vi "W07_Count.vi"() -> ()   [LabVIEW 2018]
doc: "Use this template to build a VI to use as a subVI."
panel:
  in  "stop":bool
  in  "sim read fails":bool
  in  "sim rate per s":u16
  in  "sim start":u16
  out "total this shift":u32
  out "this second":u16
  out "D202":u16
  in  "VISA resource (PLC)":refnum<visa-resource-name>
  # "FX_ReadD.vi here is a fake (W07_sub). Set sim start 65530 and sim rate 3 to see the U16 wrap."
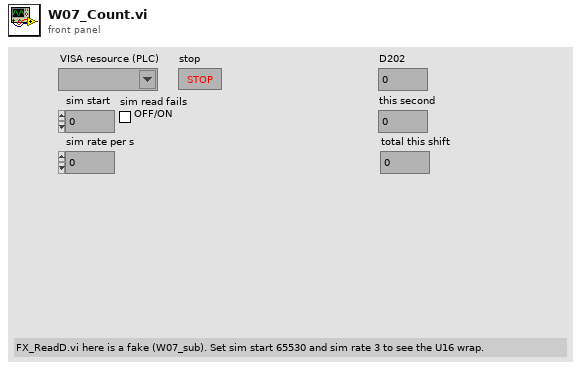
[diagram p1: front panel]
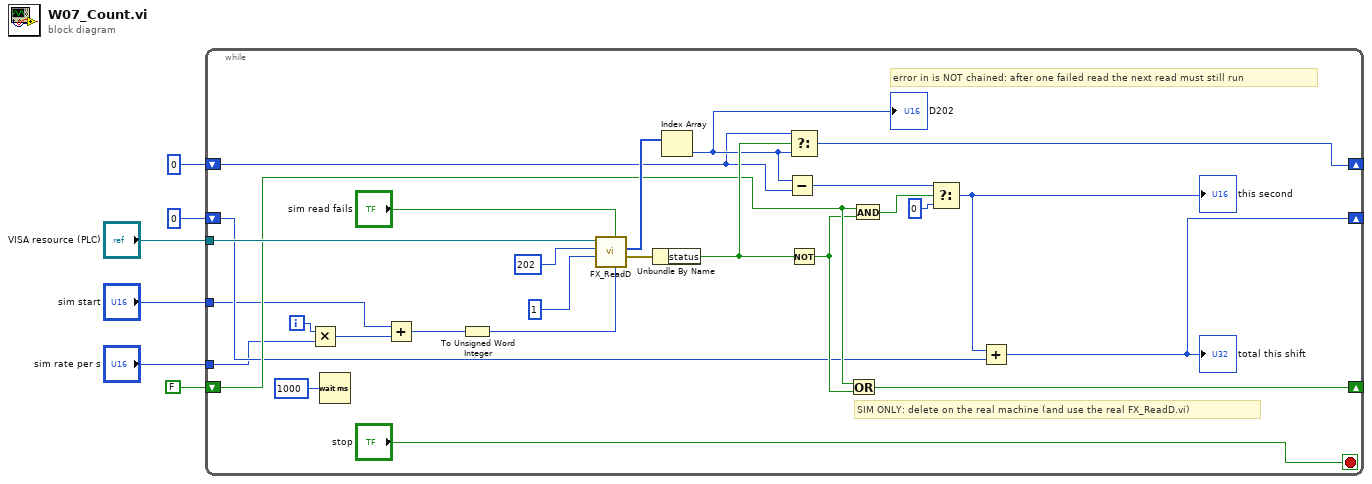
[diagram p0: block diagram]
diagram:
  n1 = while {
    tunnel: "VISA resource (PLC)" -> [w33]
    shift-right: [w25] -> _
    shift-left: u16 0 ("value (sim)") -> [w26]
    shift-right: [w22] -> _
    shift-left: FALSE -> [w24]
    shift-right: [w16] -> _
    shift-left: u32 0 ("millisecond multiple") -> [w17]
    tunnel: "sim rate per s" -> [w14]
    tunnel: "sim start" -> [w13]
    i -> [w15]
    stop <- "stop" stop-if-true
    # "error in is NOT chained: after one failed read the next read must still run"
    # "SIM ONLY: delete on the real machine (and use the real FX_ReadD.vi)"
    n2 = Multiply(x=w15, y=w14) -> (x*y=w12:i32)
    n3 = Wait (ms)(milliseconds to wait=u32 1000) -> ()  [unwired: 1 out]
    n4 = Add(x=w13, y=w12) -> (x+y=w11:i32)
    n5 = To Unsigned Word Integer(number=w11) -> (unsigned 16bit integer=w10:u16)
    n6 = call "FX_ReadD.vi"("value (sim)"=w10, "fail (sim)"="sim read fails", "Count"=u16 1, "D"=u16 202, "VISA in"=w33) -> ("error out"=w29:errorcluster, "Words"=w30:u16[])  [unwired: 4 in, 1 out]
    n7 = Unbundle By Name(w29) -> ("status"=w28:bool)
    n8 = Index Array(array=w30) -> (element=w27:u16)  [unwired: 1 in]
    "D202" <- w27
    n9 = Subtract(x=w27, y=w26) -> (x-y=w20:u16)
    n10 = Select(t=w26, s=w28, f=w27) -> (s? t:f=w25:u16)
    n11 = Not(x=w28) -> (.not. x?=w23:bool)
    n12 = Or(x=w24, y=w23) -> (x .or. y?=w22:bool)
    n13 = And(x=w24, y=w23) -> (x .and. y?=w21:bool)
    n14 = Select(t=w20, s=w21, f=u16 0) -> (s? t:f=w18:u16)
    "this second" <- w18
    n15 = Add(x=w18, y=w17) -> (x+y=w16:u32)
    "total this shift" <- w16
  }
